vi "7 segment display.vi"() -> ()   [LabVIEW 2018]
panel:
  in  "Numeric":dbl
  out "f":bool
  out "e":bool
  out "c":bool
  out "b":bool
  out "d":bool
  out "g":bool
  out "a":bool
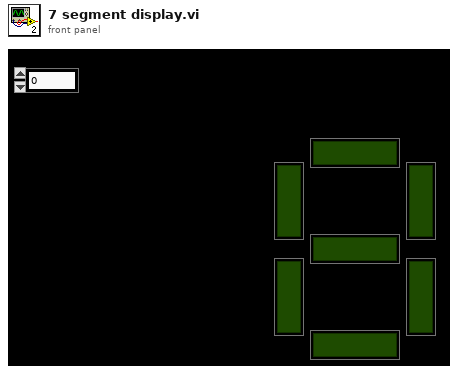
[diagram p1: front panel]
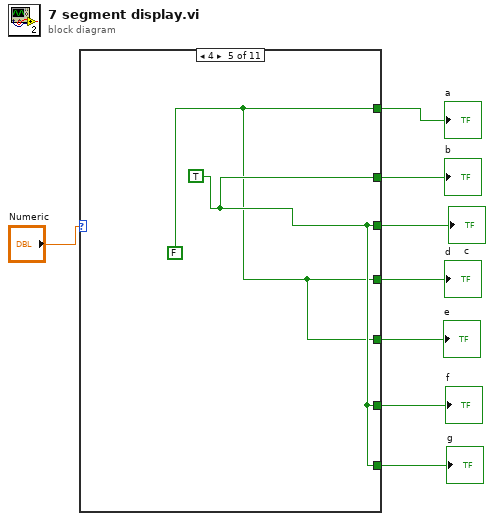
[diagram p0: block diagram]
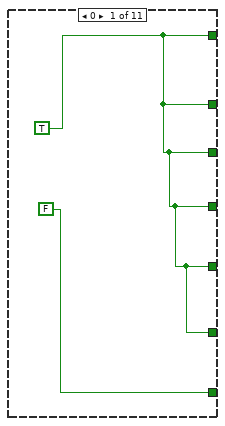
[diagram p2: hidden frame]
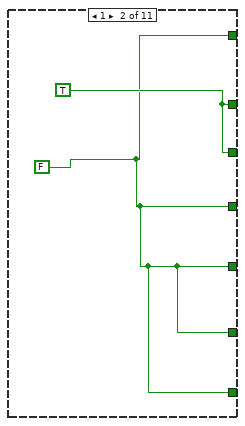
[diagram p3: hidden frame]
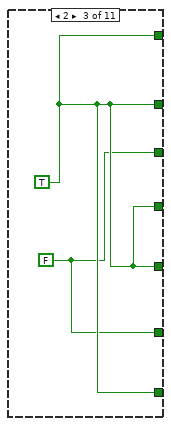
[diagram p4: hidden frame]
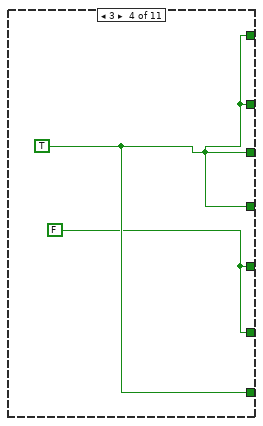
[diagram p5: hidden frame]
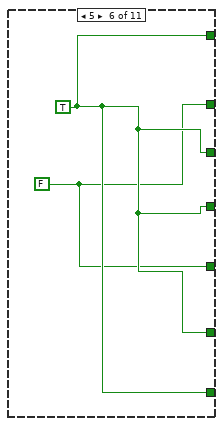
[diagram p6: hidden frame]
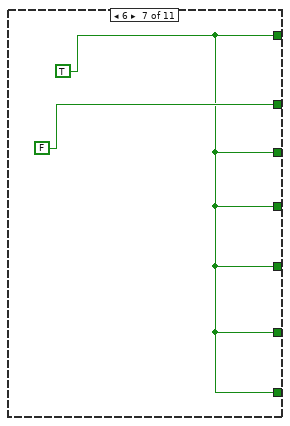
[diagram p7: hidden frame]
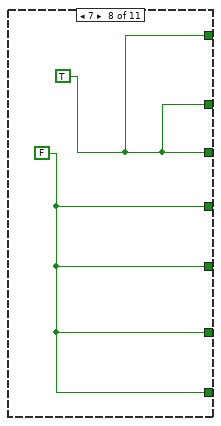
[diagram p8: hidden frame]
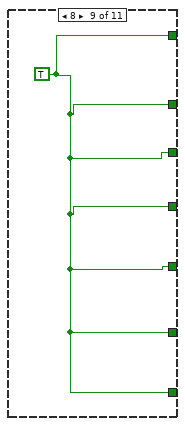
[diagram p9: hidden frame]
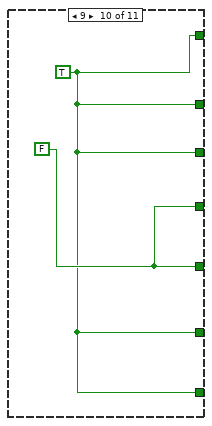
[diagram p10: hidden frame]
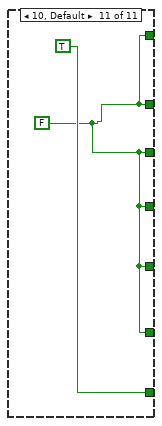
[diagram p11: hidden frame]
diagram:
  n1 = case shown="4" "Numeric" {
    tunnel: [w10 w11 w14 w16 w17 w20 w21 w24 w25 w26 w28] -> w7
    tunnel: [w10 w12 w14 w16 w18 w19 FALSE w24 w25 w26 w28] -> w6
    tunnel: [w10 w12 w13 w16 w18 w20 w21 w24 w25 w26 w28] -> w5
    tunnel: [w10 w11 w14 w16 w17 w20 w21 w23 w25 w27 w28] -> w1
    tunnel: [w10 w11 w14 w15 w17 w19 w21 w23 w25 w27 w28] -> w4
    tunnel: [w10 w11 w13 w15 w18 w20 w21 w23 w25 w26 w28] -> w3
    tunnel: [FALSE w11 w14 w16 w18 w20 w21 w23 w25 w26 TRUE] -> w2
    frame 0 {
      w10 = TRUE
    }
    frame 1 {
      w11 = FALSE
      w12 = TRUE
    }
    frame 2 {
      w13 = FALSE
      w14 = TRUE
    }
    frame 3 {
      w15 = FALSE
      w16 = TRUE
    }
    frame 4 {
      w17 = FALSE
      w18 = TRUE
    }
    frame 5 {
      w19 = FALSE
      w20 = TRUE
    }
    frame 6 {
      w21 = TRUE
    }
    frame 7 {
      w23 = FALSE
      w24 = TRUE
    }
    frame 8 {
      w25 = TRUE
    }
    frame 9 {
      w27 = FALSE
      w26 = TRUE
    }
    frame 10, Default {
      w28 = FALSE
    }
  }
  "a" <- w7
  "g" <- w2
  "d" <- w1
  "b" <- w6
  "c" <- w5
  "e" <- w4
  "f" <- w3
